vi "A_Loop.vi"(5 "Tset setting":dbl, 6 "x":dbl, 7 "N per point":i32=1, 8 "Numeric 4":dbl, 9 "Numeric 3":i32, 10 "Numeric 2":i32, 11 "Numeric":i32) -> (0 "Frequency2":string[](array[string]), 1 "Unaveraged":string[](array[string]), 2 "Frequency":string[](array[string]), 3 "Averaged":string[](array[string]), 4 "Averaged2":string[](array[string]))   [LabVIEW 2024]
panel:
  out "Progress":dbl(slide) scale=0.1..100.0
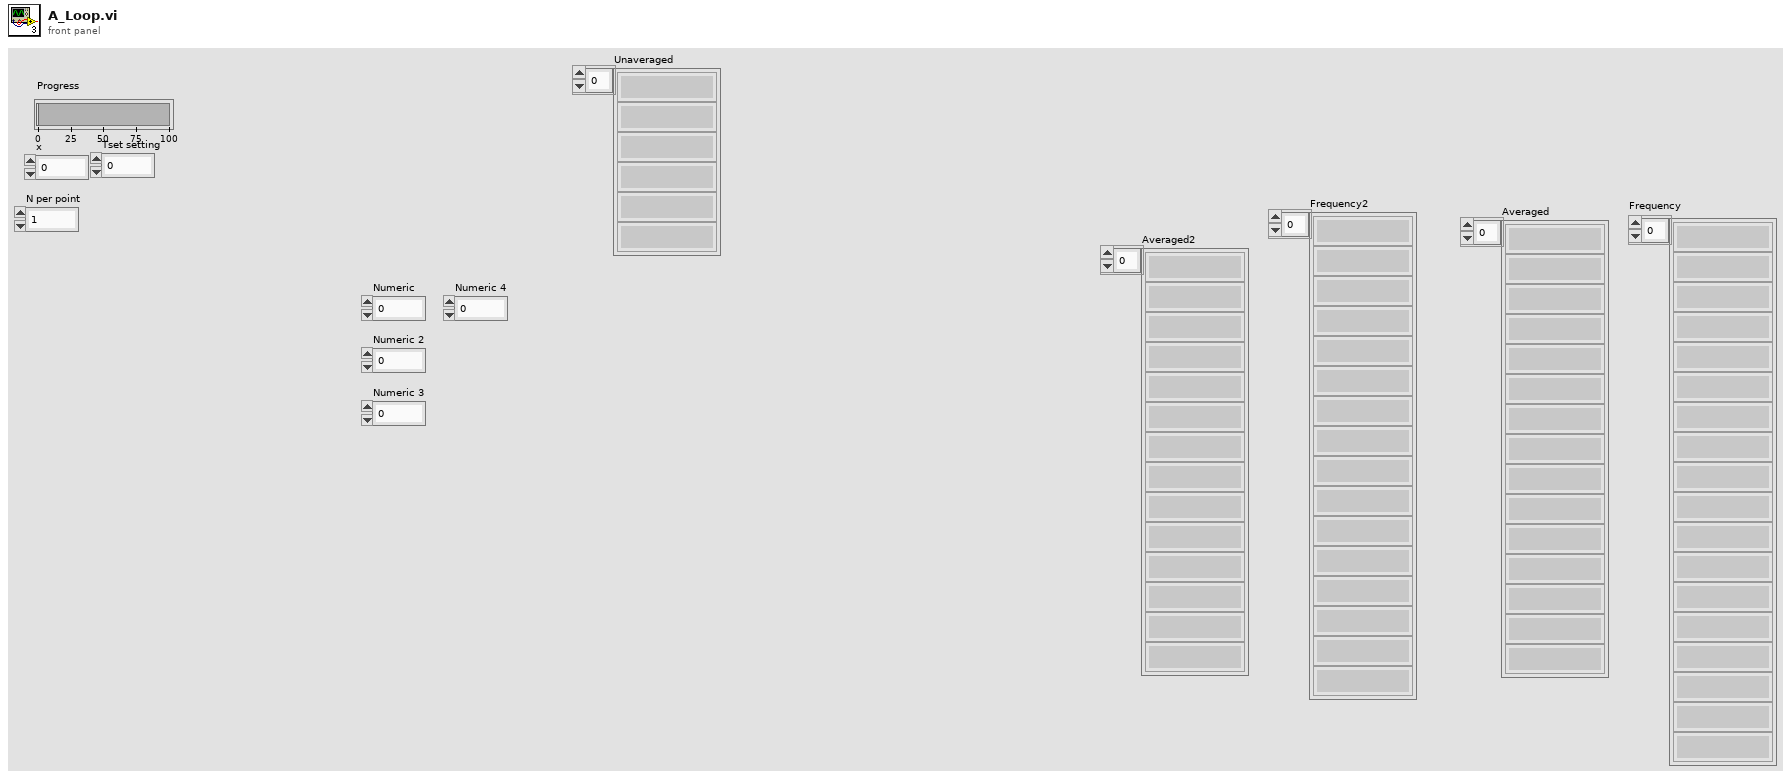
[diagram p1: front panel]
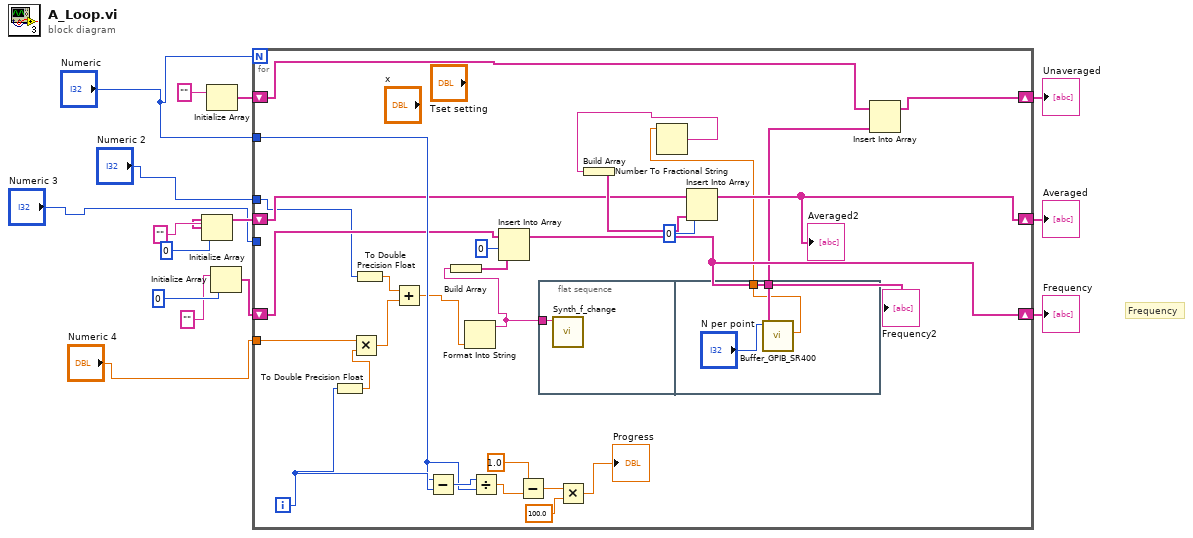
[diagram p0: block diagram]
diagram:
  # "Frequency"
  n1 = Initialize Array("", 0 ("dimension size")) -> (w11:string[])
  n2 = Initialize Array("") -> (w2:string[])  [unwired: 1 in]
  n3 = Initialize Array("", 0 ("dimension size")) -> (w10:string[])
  n4 = for {
    N: "Numeric" -> [_]
    tunnel: "Numeric 4" -> [w43]
    tunnel: "Numeric 2" -> [w20]
    tunnel: "Numeric" -> [w34]
    tunnel: "Numeric 3" -> [_]
    shift-right: [w22] -> w9
    shift-left: w11 -> [w24]
    shift-right: [w25] -> w8
    shift-left: w10 -> [w23]
    shift-right: [w18] -> w1
    shift-left: w2 -> [w19]
    i -> [w36]
    n5 = To Double Precision Float(number=w36) -> (double precision float=w42:dbl)
    n6 = Multiply(x=w43, y=w42) -> (x*y=w26:dbl)
    n7 = To Double Precision Float(number=w20) -> (double precision float=w27:dbl)
    n8 = Add(x=w27, y=w26) -> (x+y=w28:dbl)
    n9 = Subtract(x=w34, y=w36) -> (x-y=w35:i32)
    n10 = Format Into String(w28) -> (resulting string=w37:string)  [unwired: 3 in, 1 out]
    n11 = Build Array(w37) -> (w41:string[])
    n12 = Divide(x=w35, y=w34) -> (x/y=w32:dbl)
    n13 = Insert Into Array "Insert Into Array"(array=w23, index=0 ("index (row)"), new element=w41) -> (w25:string[])
    "Frequency2" <- w25
    n14 = Subtract(x=1.0, y=w32) -> (x-y=w31:dbl)
    n15 = flat-sequence {
      tunnel: w37 -> [w44]
      tunnel: [w47] -> w17
      tunnel: [w46] -> w16
      frame #0 {
        n16 = call "Synth_f_change.vi"("string"=w44) -> ()  [unwired: 11 in]
      }
      frame #1 {
        n17 = call "Buffer_GPIB_SR400.vi"("N per point"="N per point") -> ("Array"=w47:string[], "x/y"=w46:dbl)  [unwired: 9 in]
      }
    }
    n18 = Multiply(x=w31, y=100.0) -> (x*y=→"Progress":dbl)
    n19 = Number To Fractional String(number=w16) -> (F-format string=w29:string)  [unwired: 3 in]
    n20 = Build Array(w29) -> (w39:string[])
    n21 = Insert Into Array "Insert Into Array"(array=w24, index=0, new element=w39) -> (w22:string[])
    "Averaged2" <- w22
    n22 = Insert Into Array(array=w19, new element=w17) -> (w18:string[])  [unwired: 1 in]
  }
  "Averaged" <- w9
  "Frequency" <- w8
  "Unaveraged" <- w1
